vi "PLC_Test.vi"() -> ()   [LabVIEW 2018]
doc: "Use this template to build a VI to use as a subVI."
panel:
  out "error out":errorcluster
  out "Words":u16[](array[numeric])
  in  "Count":u16
  in  "Start D":u16
  in  "Value":u16
  in  "Address D":u16
  in  "Port":u16
  in  "Host":string
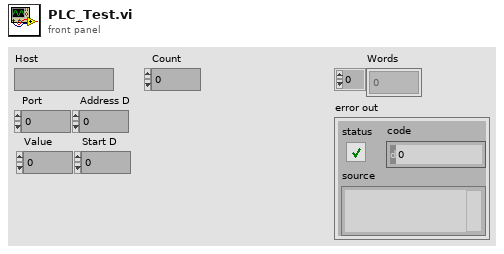
[diagram p1: front panel]
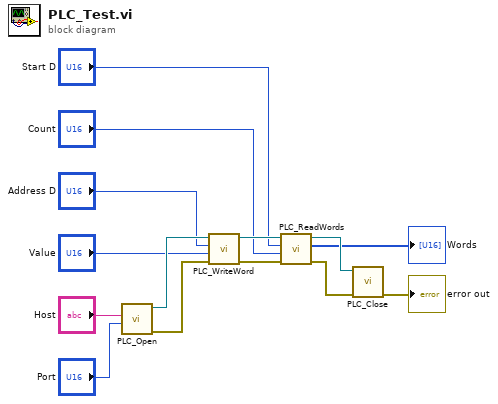
[diagram p0: block diagram]
diagram:
  n1 = call "PLC_Open.vi"("Port"="Port", "Host"="Host") -> ("error out"=w13:errorcluster, "PLC Conn"=w14:refnum<visa-resource-name>)  [unwired: 8 in]
  n2 = call "PLC_WriteWord.vi"("error in (no error)"=w13, "Value"="Value", "Address D"="Address D", "PLC Conn"=w14) -> ("error out"=w11:errorcluster, "PLC Conn out"=w12:refnum<visa-resource-name>)  [unwired: 6 in]
  n3 = call "PLC_ReadWords.vi"("error in (no error)"=w11, "Count"="Count", "Start D"="Start D", "PLC Conn"=w12) -> ("error out"=w9:errorcluster, "Words"=→"Words":u16[], "PLC Conn out"=w10:refnum<visa-resource-name>)  [unwired: 5 in]
  n4 = call "PLC_Close.vi"("error in (no error)"=w9, "PLC Conn"=w10) -> ("error out"=→"error out":errorcluster)  [unwired: 9 in]
